vi "Addon.Version.Upgrade.vi"(8 "error in (no error)":errorcluster, 11 "Device Item Ref in in":T1 format="%.0x") -> (0 "error out":errorcluster, 3 "Device Item Ref out":T1 format="%.0x")   [LabVIEW 2025, in "Diagnostics Addon Shared.lvlib"]
uses:
  Diagnostics Addon Shared.lvlib
  <vilib>/NI VeriStand/Custom Device API/Custom Device Channel Type.ctl
  <vilib>/NI VeriStand/Custom Device API/Custom Device API.lvlib
  <vilib>/NI VeriStand/Custom Device API/Custom Device Channel.ctl
  Types/Settings.Channel.ctl
  Constants.vi
  NationalInstruments.VeriStand.SystemDefinitionAPI
  <vilib>/NI/NI VeriStand Advanced SysDef API/SysDef API/Advanced System Definition.lvlib
  <vilib>/NI/NI VeriStand Advanced SysDef API/_SubVIs/SysDef.Property.Get.U32.vi
  Types/Security.Type.ctl
  <vilib>/NI/NI VeriStand Advanced SysDef API/_SubVIs/SysDef.Search.GUID.vi
  Types/Protocol.ctl
  Types/Type.ctl
  <userlib>/_OpenG.lib/lvdata/lvdata.llb/openg_variant.lvlib
  <vilib>/NI/NI VeriStand Advanced SysDef API/_SubVIs/SysDef.Property.Get.String.vi
  <vilib>/NI/NI VeriStand Advanced SysDef API/_SubVIs/SysDef.Property.Set.U32.vi
  <vilib>/NI VeriStand/Custom Device API/Custom Device Item Ref.ctl
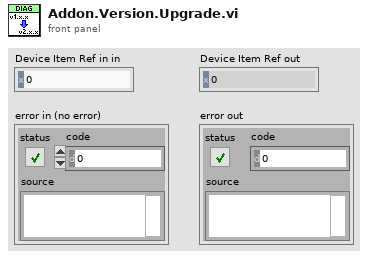
[diagram p1: front panel]
types:
  T1 = typedef "Custom Device API.lvlib/Custom Device Item Ref.ctl" = u64
  T2 = typedef "Diagnostics Addon Shared.lvlib/Security.Type.ctl" = enum16{"None", "SeedKey DLL", "MasterKey (Channel)", "MasterKey (Static)", "SeedKey DLL (Windows)"}
  T3 = typedef "Diagnostics Addon Shared.lvlib/Type.ctl" = enum16{"DID", "CDID", "PID", "CPID", "Read Memory", "Write Memory", "IO Control", "Routine Start", "Routine Request", "Routine Stop", "User Defined", "DTC Control", "Clear DTCs", "Read DTCs", "Start DTCs", "DTC Change Count", "Tester Present", "Unlock ECU", "Reset ECU", "Diag Session Control", "Communication Control", "DPID Control", "Poll Control", "Diag Comm Port Control"}
  T4 = cluster{"Name":string, "Default":i64, "Units":string, "Description":string}[]
  T5 = typedef "Custom Device API.lvlib/Custom Device Channel.ctl" = cluster{"Type":T6, "Units":string, "Default Value":dbl, "Faultable":bool, "Scalable":bool}
  T6 = typedef "Custom Device API.lvlib/Custom Device Channel Type.ctl" = enum16{"Input", "Output"}
  T7 = typedef "Diagnostics Addon Shared.lvlib/Settings.Channel.ctl" = cluster{"Name":string, "Description":string, "Channel":T5}
  T8 = typedef "Diagnostics Addon Shared.lvlib/Protocol.ctl" = enum16{"GMLAN", "KWP-2000", "UDS", "User-Defined"}
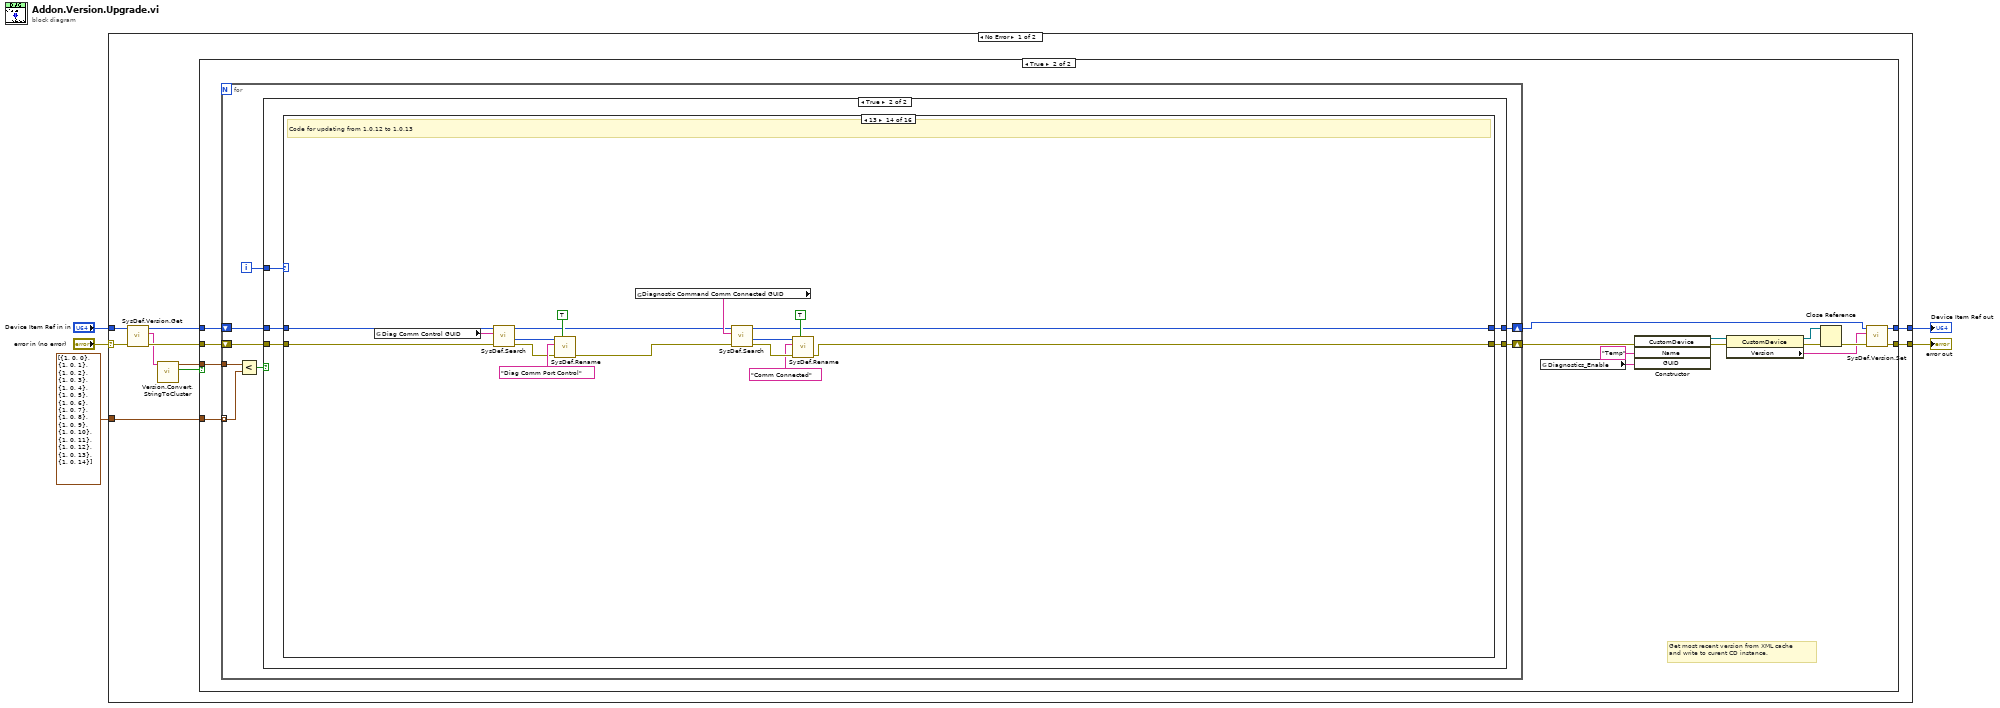
[diagram p0: block diagram]
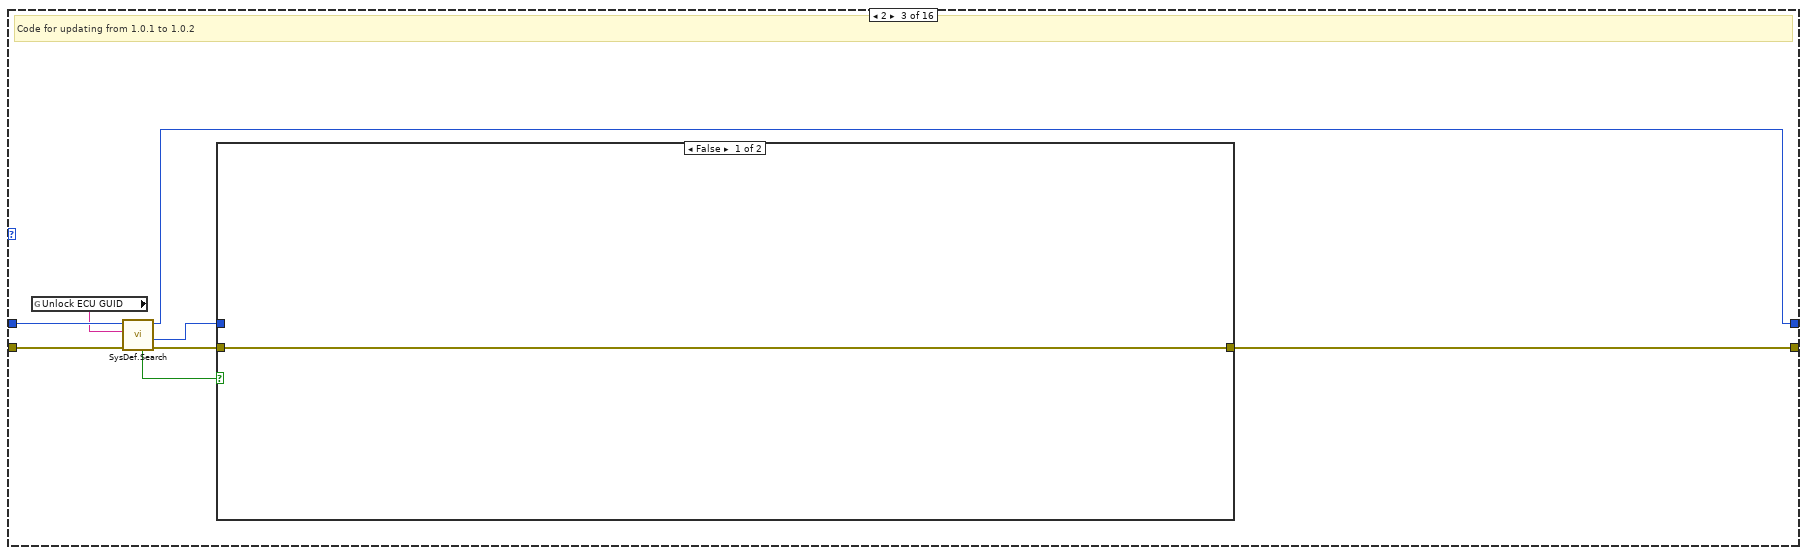
[diagram p6: hidden frame]
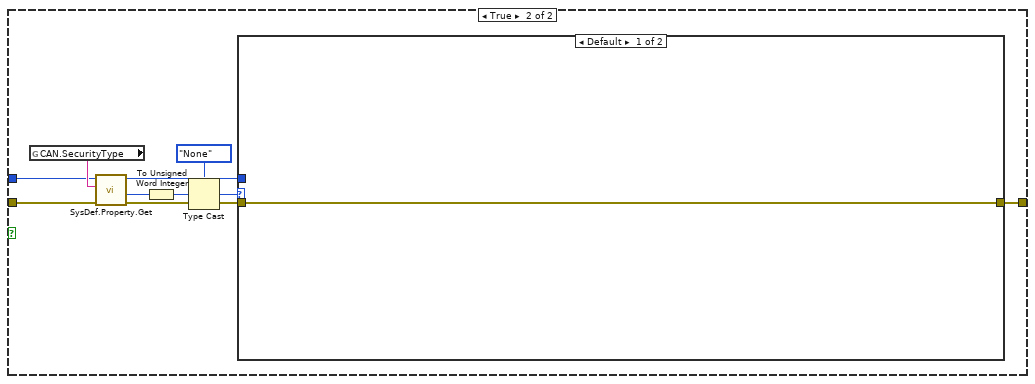
[diagram p7: hidden frame]
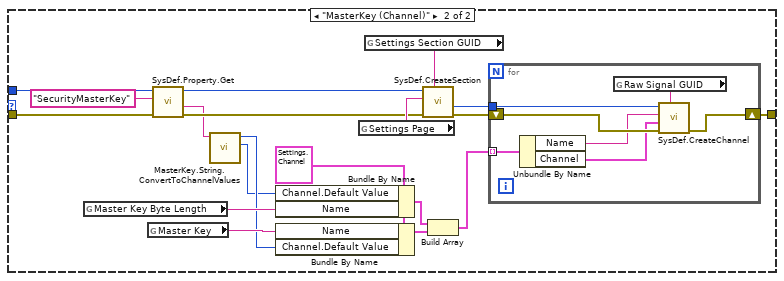
[diagram p8: hidden frame]
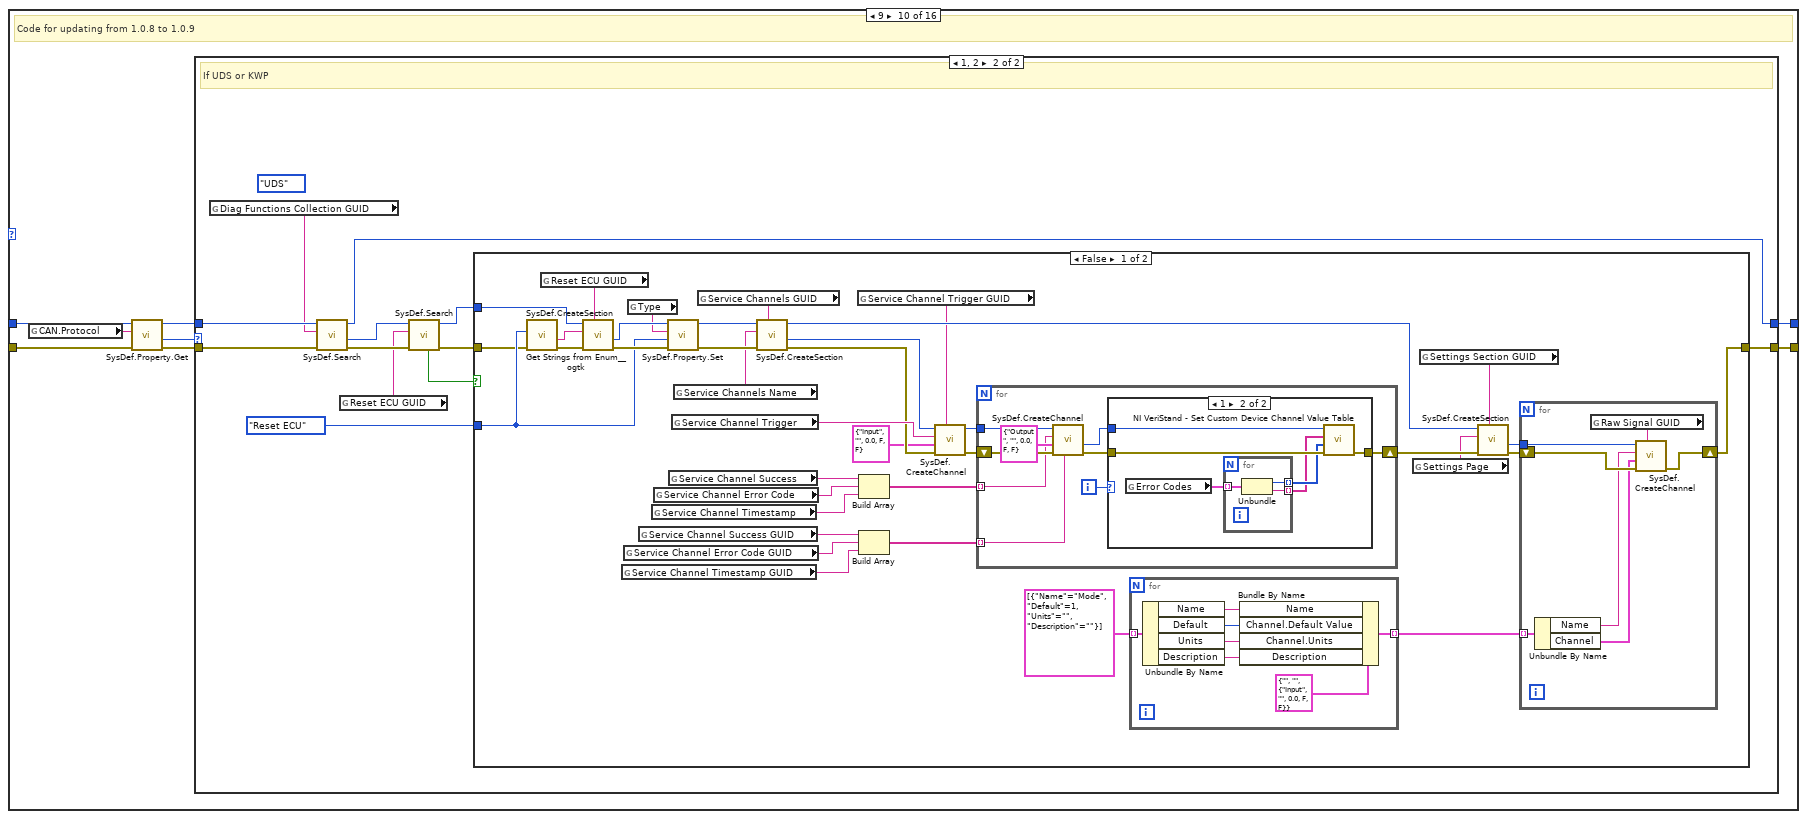
[diagram p15: hidden frame]
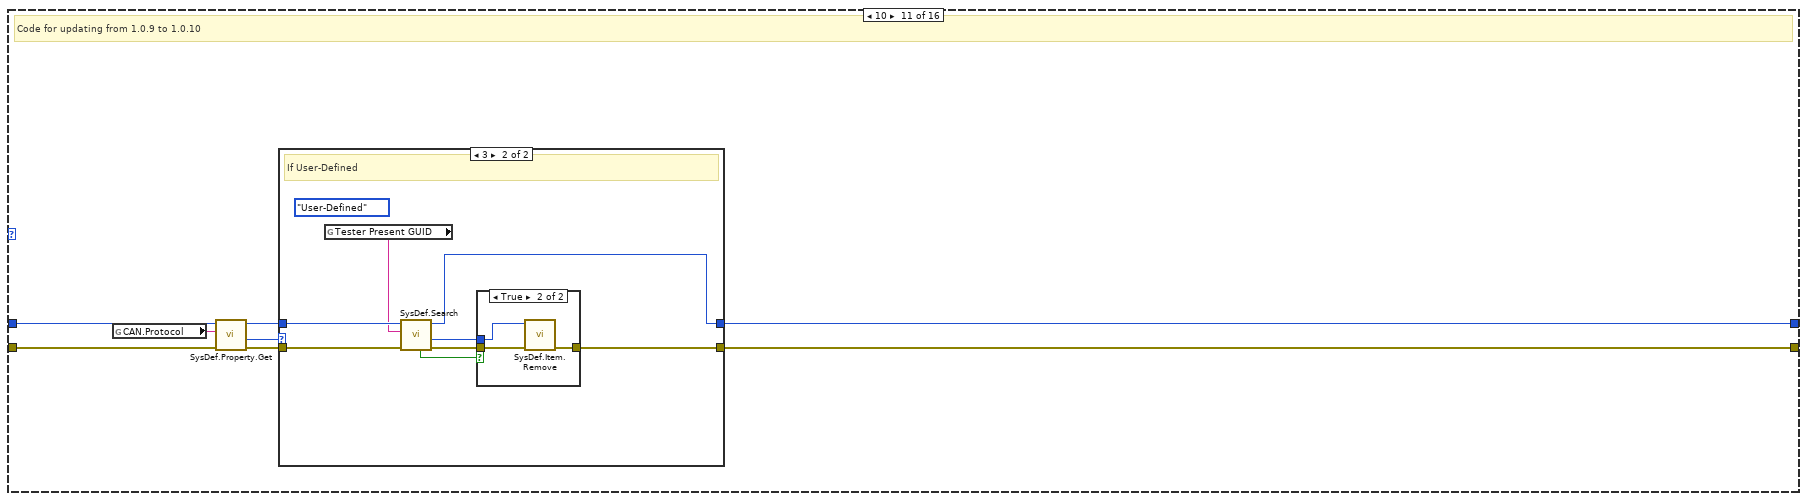
[diagram p19: hidden frame]
diagram:
  n1 = case shown="No Error" "error in (no error)" {
    selector: "error in (no error)" -> [w12 w251]
    tunnel: [w14 w251] -> w4
    tunnel: "Device Item Ref in in" -> [w11 w250]
    tunnel: [w13 w250] -> w5
    tunnel: cluster{i32, i32, i32}[] [{1, 0, 0}, {1, 0, 1}, {1, 0, 2}, {1, 0, 3}, {1, 0, 4}, {1, 0, 5}, {1, 0, 6}, {1, 0, 7}, {1, 0, 8}, {1, 0, 9}, {1, 0, 10}, {1, 0, 11}, {1, 0, 12}, {1, 0, 13}, {1, 0, 14}] -> [w15 _]
    frame No Error {
      n2 = call <vilib>:"SysDef.Version.Get.vi"("error in (no error)"=w12, "nodeID"=w11) -> ("error out"=w10:errorcluster, "Version"=w8:string, "nodeID out"=w9:u64)  [unwired: 7 in]
      n3 = call "Version.Convert.StringToCluster.vi"("Version"=w8) -> ("Version Valid?"=w6:bool, "Version"=w7:cluster{i32, i32, i32})  [unwired: 9 in]
      n4 = case shown="True" w6 {
        tunnel: w15 -> [_ w33]
        tunnel: [w17 w26] -> w14
        tunnel: [w16 w25] -> w13
        tunnel: w10 -> [w17 w20]
        tunnel: w9 -> [w16 w19]
        tunnel: w7 -> [_ w18]
        frame False {
        }
        frame True {
          # "Get most recent version from XML cache\nand write to curent CD instance."
          n5 = for {
            tunnel: w33 -> [w39] mode=indexing
            shift-right: [w41] -> w24
            shift-left: w20 -> [w35]
            shift-right: [w40] -> w23
            shift-left: w19 -> [w34]
            tunnel: w18 -> [w36]
            i -> [w37]
            n6 = Less?(x=w36, y=w39) -> (x < y?=w38:bool)
            n7 = case shown="True" w38 {
              tunnel: w35 -> [w43 w48]
              tunnel: [w43 w47] -> w41
              tunnel: w34 -> [w42 w44]
              tunnel: [w42 w45] -> w40
              tunnel: w37 -> [_ w46]
              frame False {
              }
              frame True {
                n8 = case shown="13" w46 {
                  tunnel: w48 -> [w50 w52 w60 w100 w102 w104 w106 w108 w110 w118 w206 w227 w229 w244 w247 w249]
                  tunnel: [w50 w52 w54 w100 w102 w104 w106 w108 w110 w112 w207 w227 w229 w231 w247 w249] -> w47
                  tunnel: [w49 w51 w59 w99 w101 w103 w105 w107 w109 w111 w205 w226 w228 w230 w246 w248] -> w45
                  tunnel: w44 -> [w49 w51 w58 w99 w101 w103 w105 w107 w109 w117 w204 w226 w228 w243 w246 w248]
                  frame 0 {
                    # "Initial Onload"
                  }
                  frame 1 {
                    # "Code for updating from 1.0.0 to 1.0.1"
                  }
                  frame 2 {
                    # "Code for updating from 1.0.1 to 1.0.2"
                    n9 = global read "Constants.vi" "Unlock ECU GUID"() -> (w53:string)
                    n10 = call-poly <vilib>:"SysDef.Search.vi"("error in (no error)"=w60, "GUID"=w53, "nodeID"=w58) -> ("error out"=w56:errorcluster, "Value out"=w55:u64, "nodeID out"=w59:u64, "Found?"=w57:bool)  [unwired: 5 in]
                    n11 = case shown="False" w57 {
                      tunnel: w56 -> [w61 w66]
                      tunnel: w55 -> [_ w69]
                      tunnel: [w61 w71] -> w54
                      frame False {
                      }
                      frame True {
                        n12 = global read "Constants.vi" "CAN.SecurityType"() -> (w70:string)
                        n13 = call-poly <vilib>:"SysDef.Property.Get.vi"("error in (no error)"=w66, "Property Name"=w70, "nodeID"=w69) -> ("error out"=w67:errorcluster, "Value out"=w65:u32, "nodeID out"=w68:u64)  [unwired: 5 in, 1 out]
                        n14 = To Unsigned Word Integer(number=w65) -> (unsigned 16bit integer=w64:u16)
                        n15 = Type Cast(type=Security.Type."None" ("Type"), x=w64) -> (*(type *) &x=w62:T2)
                        n16 = case shown="Default" w62 {
                          tunnel: w67 -> [w72 w85]
                          tunnel: w68 -> [_ w84]
                          tunnel: [w72 w77] -> w71
                          frame Default {
                          }
                          frame "MasterKey (Channel)" {
                            w87 = T7 {"Name"="Byte Length", "Description"="", "Channel"={"Type"=enum."Input", "Units"="", "Default Value"=0.0, "Faultable"=FALSE, "Scalable"=FALSE}} ("cluster")
                            n17 = global read "Constants.vi" "Master Key Byte Length"() -> (w89:string)
                            n18 = global read "Constants.vi" "Master Key"() -> (w88:string)
                            n19 = call-poly <vilib>:"SysDef.Property.Get.vi"("error in (no error)"=w85, "Property Name"="SecurityMasterKey" ("CAN.SecurityMasterKey"), "nodeID"=w84) -> ("error out"=w79:errorcluster, "Value out"=w76:string, "nodeID out"=w78:u64)  [unwired: 5 in, 1 out]
                            n20 = call "MasterKey.String.ConvertToChannelValues.vi"("Master Key"=w76) -> ("Length"=w73:i32, "Value"=w74:u64)  [unwired: 9 in]
                            n21 = Bundle By Name(cluster=w87, "Channel.Default Value"=w73, "Name"=w89) -> (w90:T7)
                            n22 = Bundle By Name(cluster=w87, "Name"=w88, "Channel.Default Value"=w74) -> (w91:T7)
                            n23 = global read "Constants.vi" "Settings Page"() -> (w83:string)
                            n24 = global read "Constants.vi" "Settings Section GUID"() -> (w82:string)
                            n25 = call <vilib>:"SysDef.CreateSection.vi"("GUID"=w82, "error in (no error)"=w79, "Name"=w83, "nodeID"=w78) -> ("error out"=w80:errorcluster, "New NodeID"=w81:u64)  [unwired: 4 in, 2 out]
                            n26 = Build Array(w90, w91) -> (w75:T7[])
                            n27 = for {
                              tunnel: w81 -> [w96]
                              shift-right: [w95] -> w77
                              shift-left: w80 -> [w97]
                              tunnel: w75 -> [w92] mode=indexing
                              n28 = Unbundle By Name(w92) -> ("Name"=w94:string, "Channel"=w93:T5)
                              n29 = global read "Constants.vi" "Raw Signal GUID"() -> (w98:string)
                              n30 = call <vilib>:"SysDef.CreateChannel.vi"("GUID"=w98, "error in (no error)"=w97, "Channel"=w93, "Name"=w94, "nodeID"=w96) -> ("error out"=w95:errorcluster)  [unwired: 3 in, 3 out]
                            }
                          }
                        }
                      }
                    }
                  }
                  frame 3 {
                    # "Code for updating from 1.0.2 to 1.0.3"
                  }
                  frame 4 {
                    # "Code for updating from 1.0.3 to 1.0.4"
                  }
                  frame 5 {
                    # "Code for updating from 1.0.4 to 1.0.5"
                  }
                  frame 6 {
                    # "Code for updating from 1.0.5 to 1.0.6"
                  }
                  frame 7 {
                    # "Code for updating from 1.0.6 to 1.0.7"
                  }
                  frame 8 {
                    # "Code for updating from 1.0.7 to 1.0.8"
                  }
                  frame 9 {
                    # "Code for updating from 1.0.8 to 1.0.9"
                    n31 = global read "Constants.vi" "CAN.Protocol"() -> (w116:string)
                    n32 = call-poly <vilib>:"SysDef.Property.Get.vi"("error in (no error)"=w118, "Property Name"=w116, "nodeID"=w117) -> ("error out"=w113:errorcluster, "Value out"=w115:u32, "nodeID out"=w114:u64)  [unwired: 5 in, 1 out]
                    n33 = case shown="1, 2" w115 {
                      tunnel: w114 -> [w119 w132]
                      tunnel: w113 -> [w120 w131]
                      tunnel: [w120 w125] -> w112
                      tunnel: [w119 w124] -> w111
                      frame 0, Default {
                      }
                      frame 1, 2 {
                        (unwired) Protocol."UDS" ("Diagnostic Protocol")
                        # "If UDS or KWP"
                        n34 = global read "Constants.vi" "Diag Functions Collection GUID"() -> (w130:string)
                        n35 = call-poly <vilib>:"SysDef.Search.vi"("error in (no error)"=w131, "GUID"=w130, "nodeID"=w132) -> ("error out"=w128:errorcluster, "Value out"=w129:u64, "nodeID out"=w124:u64)  [unwired: 5 in, 1 out]
                        n36 = global read "Constants.vi" "Reset ECU GUID"() -> (w121:string)
                        n37 = call-poly <vilib>:"SysDef.Search.vi"("error in (no error)"=w128, "GUID"=w121, "nodeID"=w129) -> ("error out"=w126:errorcluster, "nodeID out"=w122:u64, "Found?"=w127:bool)  [unwired: 5 in, 1 out]
                        n38 = case shown="False" w127 {
                          tunnel: w126 -> [w135 w203]
                          tunnel: [w133 w203] -> w125
                          tunnel: Type."Reset ECU" ("Type") -> [w136 _]
                          tunnel: w122 -> [w134 _]
                          frame False {
                            n39 = call <userlib>:"Get Strings from Enum__ogtk.vi"("error in (no error)"=w135, "Enum"=w136) -> ("error out"=w140:errorcluster, "String Value"=w139:string)  [unwired: 6 in, 2 out]
                            n40 = global read "Constants.vi" "Reset ECU GUID"() -> (w141:string)
                            n41 = call <vilib>:"SysDef.CreateSection.vi"("GUID"=w141, "error in (no error)"=w140, "Name"=w139, "nodeID"=w134) -> ("error out"=w143:errorcluster, "New NodeID"=w144:u64)  [unwired: 4 in, 2 out]
                            n42 = global read "Constants.vi" "Service Channel Timestamp GUID"() -> (w156:string)
                            n43 = global read "Constants.vi" "Service Channel Error Code GUID"() -> (w155:string)
                            n44 = global read "Constants.vi" "Type"() -> (w142:string)
                            n45 = global read "Constants.vi" "Service Channel Success GUID"() -> (w157:string)
                            n46 = global read "Constants.vi" "Service Channel Timestamp"() -> (w151:string)
                            n47 = global read "Constants.vi" "Service Channel Error Code"() -> (w152:string)
                            n48 = call-poly <vilib>:"SysDef.Property.Set.vi"("error in (no error)"=w143, "Value"=w136, "Property Name"=w142, "nodeID"=w144) -> ("error out"=w161:errorcluster, "nodeID out"=w162:u64)  [unwired: 6 in]
                            n49 = global read "Constants.vi" "Service Channel Success"() -> (w153:string)
                            n50 = global read "Constants.vi" "Service Channel Trigger"() -> (w148:string)
                            n51 = global read "Constants.vi" "Service Channels Name"() -> (w150:string)
                            n52 = global read "Constants.vi" "Service Channels GUID"() -> (w149:string)
                            n53 = call <vilib>:"SysDef.CreateSection.vi"("GUID"=w149, "error in (no error)"=w161, "Name"=w150, "nodeID"=w162) -> ("error out"=w146:errorcluster, "New NodeID"=w145:u64, "nodeID out"=w167:u64)  [unwired: 4 in, 1 out]
                            n54 = global read "Constants.vi" "Service Channel Trigger GUID"() -> (w147:string)
                            n55 = Build Array(w153, w152, w151) -> (w154:string[])
                            n56 = Build Array(w157, w155, w156) -> (w158:string[])
                            n57 = call <vilib>:"SysDef.CreateChannel.vi"("GUID"=w147, "error in (no error)"=w146, "Channel"=T5 {"Type"=enum."Input", "Units"="", "Default Value"=0.0, "Faultable"=FALSE, "Scalable"=FALSE}, "Name"=w148, "nodeID"=w145) -> ("error out"=w160:errorcluster, "nodeID out"=w159:u64)  [unwired: 3 in, 2 out]
                            n58 = for {
                              tunnel: w159 -> [w190]
                              shift-right: [w185] -> w168
                              shift-left: w160 -> [w191]
                              tunnel: w154 -> [w189] mode=indexing
                              tunnel: w158 -> [w184] mode=indexing
                              i -> [w188]
                              n59 = call <vilib>:"SysDef.CreateChannel.vi"("GUID"=w184, "error in (no error)"=w191, "Channel"=T5 {"Type"=enum."Output", "Units"="", "Default Value"=0.0, "Faultable"=FALSE, "Scalable"=FALSE}, "Name"=w189, "nodeID"=w190) -> ("error out"=w187:errorcluster, "New NodeID"=w186:u64)  [unwired: 3 in, 2 out]
                              n60 = case shown="1" w188 {
                                tunnel: w187 -> [w193 w198]
                                tunnel: w186 -> [_ w199]
                                tunnel: [w193 w197] -> w185
                                frame 0, Default {
                                }
                                frame 1 {
                                n61 = global read "Constants.vi" "Error Codes"() -> (w196:cluster{"Code":i32, "String":string}[])
                                n62 = for {
                                tunnel: w196 -> [w202] mode=indexing
                                tunnel: [w201] -> w195 mode=indexing
                                tunnel: [w200] -> w194 mode=indexing
                                n63 = Unbundle(w202) -> ("Code"=w201:i32, "String"=w200:string)
                                }
                                n64 = call <vilib>:"NI VeriStand - Set Custom Device Channel Value Table.vi"("error in (no error)"=w198, "Values"=w195, "Names"=w194, "Channel Ref in"=w199) -> ("error out"=w197:errorcluster)  [unwired: 6 in, 1 out]
                                }
                              }
                            }
                            n65 = for {
                              tunnel: T4 [{"Name"="Mode", "Default"=1, "Units"="", "Description"=""}] -> [w182] mode=indexing
                              tunnel: [w178] -> w169 mode=indexing
                              n66 = Unbundle By Name(w182) -> ("Name"=w181:string, "Default"=w180:i64, "Units"=w179:string, "Description"=w177:string)
                              n67 = Bundle By Name(cluster=T7 {"Name"="", "Description"="", "Channel"={"Type"=enum."Input", "Units"="", "Default Value"=0.0, "Faultable"=FALSE, "Scalable"=FALSE}}, "Name"=w181, "Channel.Default Value"=w180, "Channel.Units"=w179, "Description"=w177) -> (w178:T7)
                            }
                            n68 = global read "Constants.vi" "Settings Page"() -> (w163:string)
                            n69 = global read "Constants.vi" "Settings Section GUID"() -> (w164:string)
                            n70 = call <vilib>:"SysDef.CreateSection.vi"("GUID"=w164, "error in (no error)"=w168, "Name"=w163, "nodeID"=w167) -> ("error out"=w166:errorcluster, "New NodeID"=w165:u64)  [unwired: 4 in, 2 out]
                            n71 = for {
                              tunnel: w165 -> [w174]
                              shift-right: [w173] -> w133
                              shift-left: w166 -> [w175]
                              tunnel: w169 -> [w172] mode=indexing
                              n72 = Unbundle By Name(w172) -> ("Name"=w171:string, "Channel"=w170:T5)
                              n73 = global read "Constants.vi" "Raw Signal GUID"() -> (w176:string)
                              n74 = call <vilib>:"SysDef.CreateChannel.vi"("GUID"=w176, "error in (no error)"=w175, "Channel"=w170, "Name"=w171, "nodeID"=w174) -> ("error out"=w173:errorcluster)  [unwired: 3 in, 3 out]
                            }
                          }
                          frame True {
                          }
                        }
                      }
                    }
                  }
                  frame 10 {
                    # "Code for updating from 1.0.9 to 1.0.10"
                    n75 = global read "Constants.vi" "CAN.Protocol"() -> (w211:string)
                    n76 = call-poly <vilib>:"SysDef.Property.Get.vi"("error in (no error)"=w206, "Property Name"=w211, "nodeID"=w204) -> ("error out"=w208:errorcluster, "Value out"=w210:u32, "nodeID out"=w209:u64)  [unwired: 5 in, 1 out]
                    n77 = case shown="3" w210 {
                      tunnel: w209 -> [w212 w221]
                      tunnel: w208 -> [w213 w220]
                      tunnel: [w213 w215] -> w207
                      tunnel: [w212 w216] -> w205
                      frame 0, Default {
                      }
                      frame 3 {
                        (unwired) Protocol."User-Defined" ("Diagnostic Protocol")
                        # "If User-Defined"
                        n78 = global read "Constants.vi" "Tester Present GUID"() -> (w219:string)
                        n79 = call-poly <vilib>:"SysDef.Search.vi"("error in (no error)"=w220, "GUID"=w219, "nodeID"=w221) -> ("error out"=w217:errorcluster, "Value out"=w218:u64, "nodeID out"=w216:u64, "Found?"=w214:bool)  [unwired: 5 in]
                        n80 = case shown="True" w214 {
                          tunnel: w218 -> [_ w225]
                          tunnel: w217 -> [w222 w224]
                          tunnel: [w222 w223] -> w215
                          frame False {
                          }
                          frame True {
                            n81 = call <vilib>:"SysDef.Item.Remove.vi"("error in (no error)"=w224, "nodeID"=w225) -> ("error out"=w223:errorcluster)  [unwired: 8 in, 1 out]
                          }
                        }
                      }
                    }
                  }
                  frame 11 {
                    # "Code for updating from 1.0.10 to 1.0.11"
                  }
                  frame 12 {
                    # "Code for updating from 1.0.11 to 1.0.12"
                  }
                  frame 13 {
                    # "Code for updating from 1.0.12 to 1.0.13"
                    n82 = global read "Constants.vi" "Diag Comm Control GUID"() -> (w245:string)
                    n83 = call-poly <vilib>:"SysDef.Search.vi"("error in (no error)"=w244, "GUID"=w245, "nodeID"=w243) -> ("error out"=w239:errorcluster, "Value out"=w242:u64, "nodeID out"=w232:u64)  [unwired: 5 in, 1 out]
                    n84 = call <vilib>:"SysDef.Rename.vi"("Force Rename (F)"=TRUE, "error in (no error)"=w239, "Name"="Diag Comm Port Control" ("Enum Name"), "nodeID"=w242) -> ("error out"=w234:errorcluster)  [unwired: 5 in, 2 out]
                    n85 = global read "Constants.vi" "Diagnostic Command Comm Connected GUID"() -> (w235:string)
                    n86 = call-poly <vilib>:"SysDef.Search.vi"("error in (no error)"=w234, "GUID"=w235, "nodeID"=w232) -> ("error out"=w238:errorcluster, "Value out"=w236:u64, "nodeID out"=w230:u64)  [unwired: 5 in, 1 out]
                    n87 = call <vilib>:"SysDef.Rename.vi"("Force Rename (F)"=TRUE, "error in (no error)"=w238, "Name"="Comm Connected" ("Diagnostic Command Comm Connected"), "nodeID"=w236) -> ("error out"=w231:errorcluster)  [unwired: 5 in, 2 out]
                  }
                  frame 14 {
                    # "Code for updating from 1.0.13 to 1.0.14"
                  }
                  frame Default {
                    # "Nothing to update"
                  }
                }
              }
            }
          }
          n88 = global read "Constants.vi" "Diagnostics_Enable"() -> (w21:string)
          n89 = constructor class="CustomDevice"(error in=w24, "Name"="Temp", "GUID"=w21) -> (reference out=w32:refnum<k24>, error out=w31:errorcluster)  [unwired: 2 in, 3 out]
          n90 = property class="CustomDevice"(reference=w32, error in=w31) -> (reference out=w29:refnum<k24>, error out=w30:errorcluster, "Version"=w27:string)
          n91 = Close Reference(reference=w29, error in (no error)=w30) -> (error out=w28:errorcluster)
          n92 = call <vilib>:"SysDef.Version.Set.vi"("error in (no error)"=w28, "Version"=w27, "nodeID"=w23) -> ("error out"=w26:errorcluster, "nodeID out"=w25:u64)  [unwired: 7 in]
        }
      }
    }
    frame Error {
    }
  }
  "Device Item Ref out" <- w5
  "error out" <- w4
